vi "test2.vi"() -> ()   [LabVIEW 2017]
uses:
  <userlib>/_NEVSTOP/Communicable State Machine(CSM)/AdvanceAPI/CSM - Revert Arguments-Safe String.vi
  <userlib>/_NEVSTOP/Communicable State Machine(CSM)/_Shared/Trim Single-line Text.vi
  <userlib>/_NEVSTOP/Communicable State Machine(CSM)/AdvanceAPI/CSM - Make String Arguments Safe.vi
  <userlib>/_NEVSTOP/Communicable State Machine(CSM)/AdvanceAPI/CSM - Break Down Multiple States String.vi
  <userlib>/_NEVSTOP/Communicable State Machine(CSM)/AdvanceAPI/CSM - Compact Multiple States.vi
  <userlib>/_NEVSTOP/Communicable State Machine(CSM)/AdvanceAPI/CSM - Keywords.vi
  <userlib>/_NEVSTOP/Communicable State Machine(CSM)/_Polymophic/CSM - Filter Duplicated Lines.vi
  <userlib>/_NEVSTOP/Communicable State Machine(CSM)/Communicable State Machine.lvlib
  ad7296c1-f9ce-49fc-bda0-69987307e577.vi
  bdc5c617-8b58-41cb-8bd3-c5aaa467307a.vi
  <userlib>/_NEVSTOP/Communicable State Machine(CSM)/addons/MassData-Parameter/CSM MassData Parameter Support.lvlib
  <userlib>/_NEVSTOP/Communicable State Machine(CSM)/_Polymophic/Build No-Reply Asynchronous Message with Arguments.vi
panel:
  out "Found":bool
  out "Waited(ms) 2":u32
  out "Waited(ms)":u32
  out "error out":errorcluster
  out "A 4":bool=TRUE
  in  "停止":bool
  in  "布尔":bool
  out "A 3":bool=TRUE
  out "A 2":bool=TRUE
  out "A 1":bool=TRUE
  out "Error Occurred":errorcluster
  out "State History":string
  in  "Name (\"\" to Use UUID)":string="test2"
  in  "Slide":dbl(slide) caption="Flood of Events:\n\nPanel/Pane Size Event\nSlide/Knob... User Event by dragging\nNumeric Control Value Change Event by Arraw Button" scale=0.0..10.0
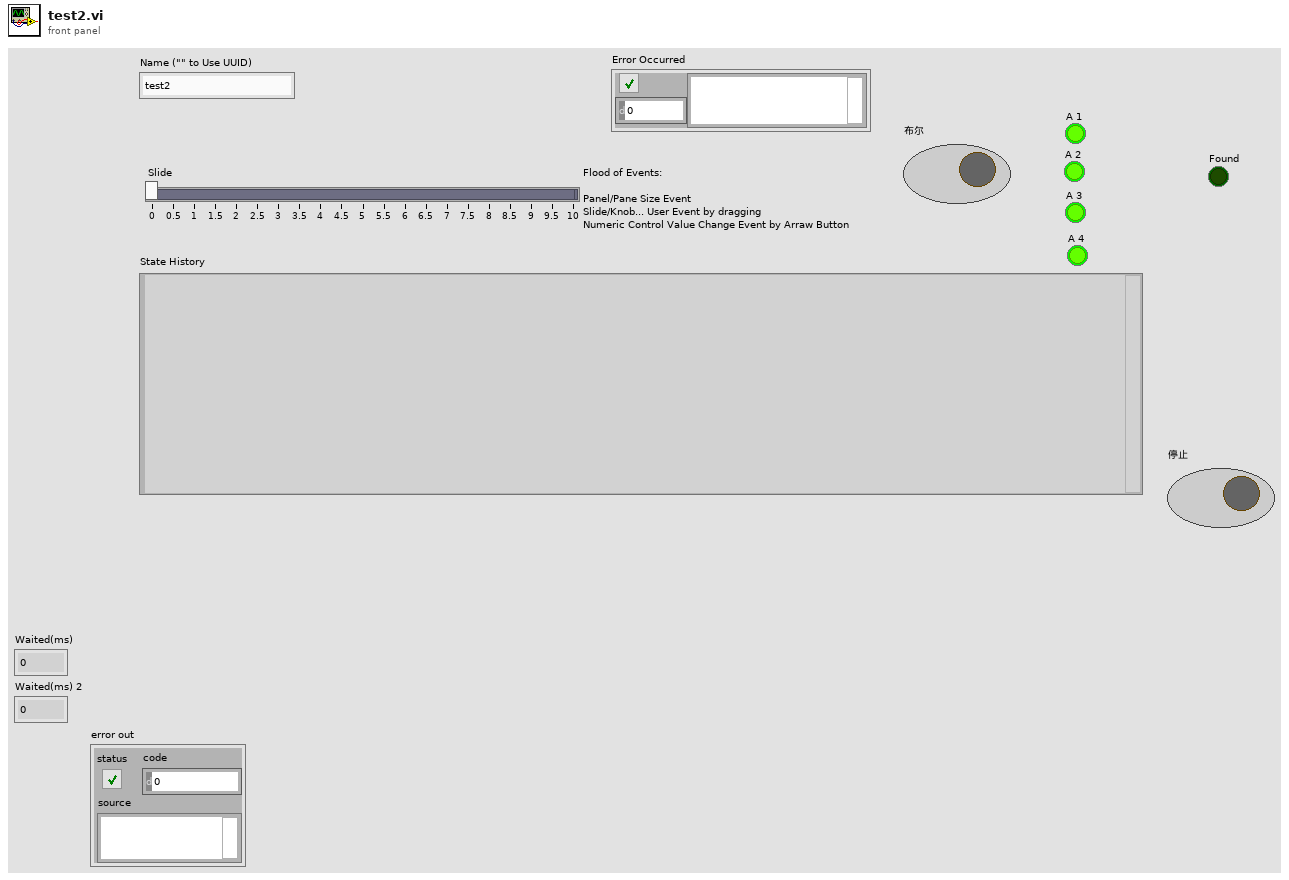
[diagram p1: front panel]
types:
  T1 = enum32{"Invalid", "Standard", "Closed", "Hidden", "Minimized", "Maximized"}
  T2 = enum32{"invalid app kind", "Development System", "Run Time System", "Student Edition", "Embedded LabVIEW", "Evaluation", "Custom"}
  T3 = typedef "Communicable State Machine.lvlib/_CSM_Response Source Message.ctl" = cluster{"‘State":string, "’Arguments":string, "’Error":errorcluster}
  T4 = cluster{"Current VI Reference":refnum<vi>, "Close Panel on Exit?":bool}
  T5 = cluster{"Core":cluster{"Current VI Reference":refnum<vi>, "Close Panel on Exit?":bool}, "Your Boolean data":bool, "Your string data":string}
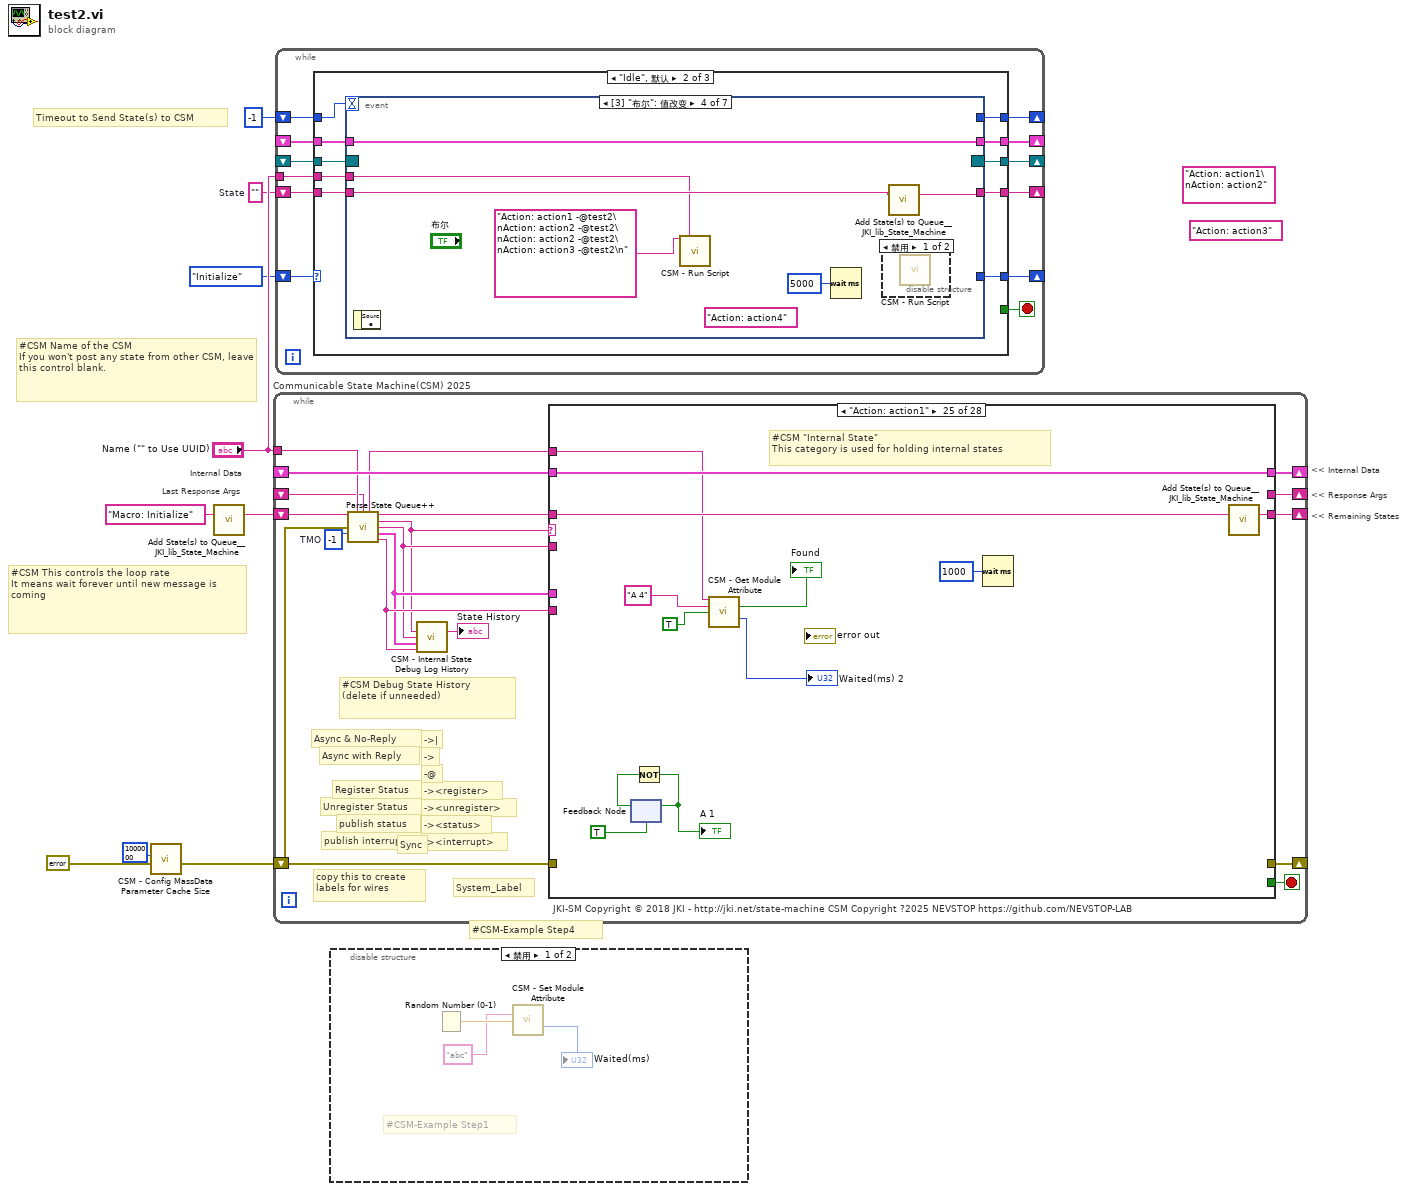
[diagram p0: block diagram]
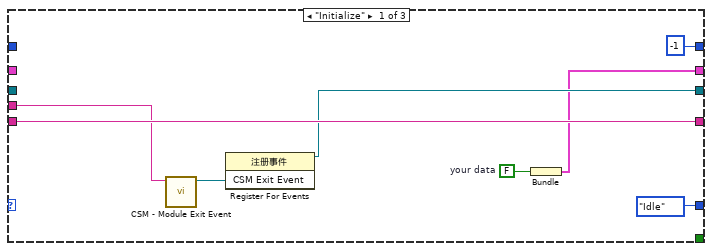
[diagram p3: hidden frame]
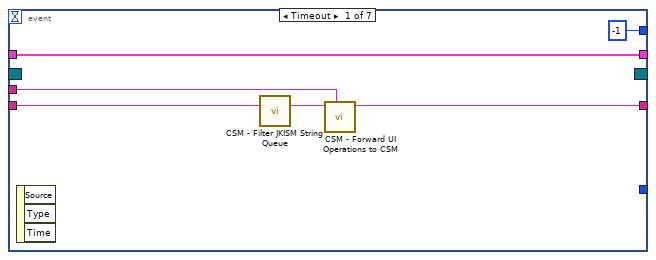
[diagram p4: hidden frame]
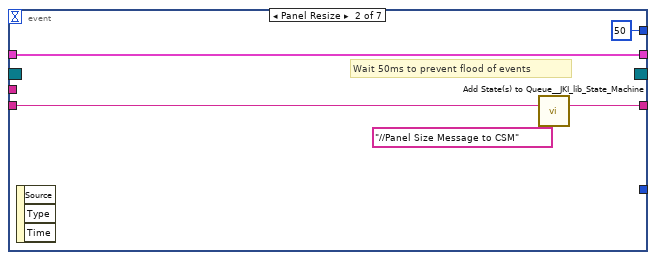
[diagram p5: hidden frame]
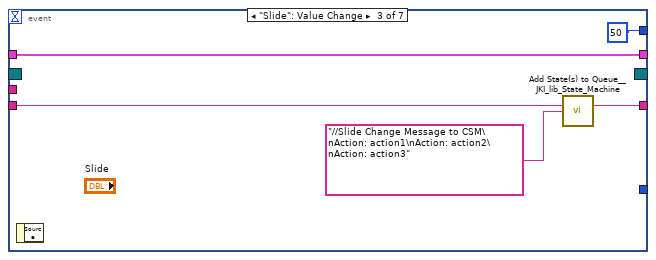
[diagram p6: hidden frame]
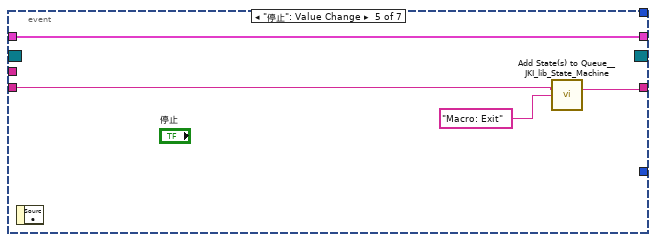
[diagram p8: hidden frame]
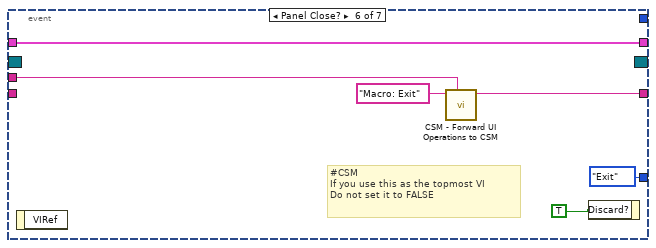
[diagram p9: hidden frame]
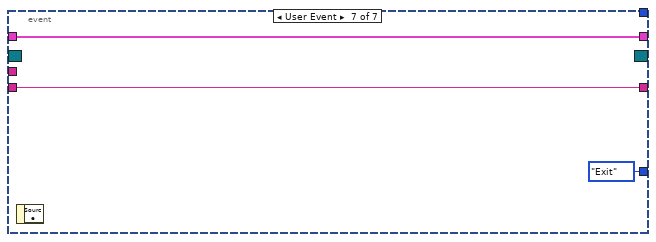
[diagram p10: hidden frame]
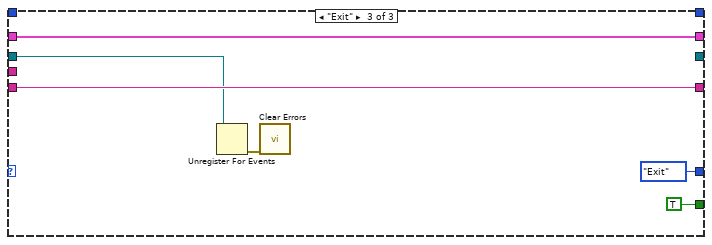
[diagram p11: hidden frame]
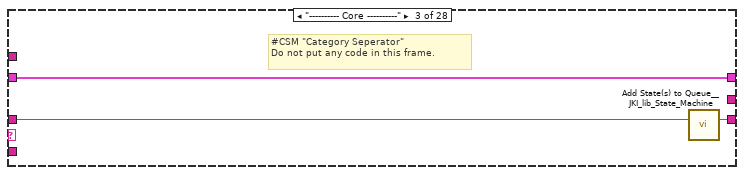
[diagram p14: hidden frame]
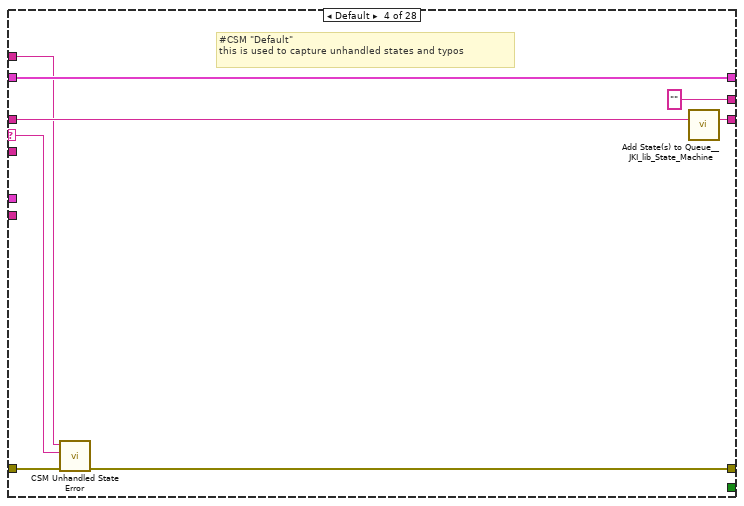
[diagram p15: hidden frame]
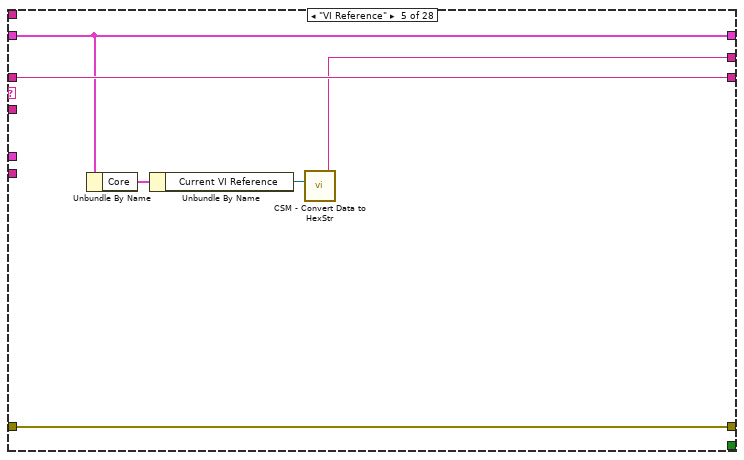
[diagram p16: hidden frame]
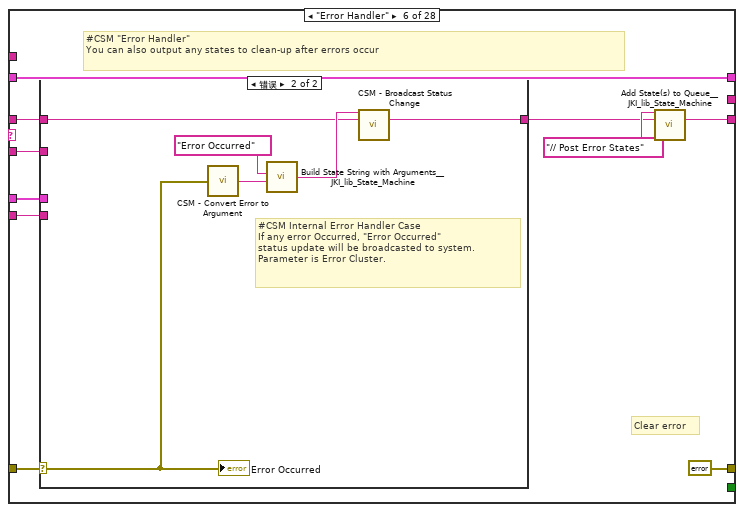
[diagram p17: hidden frame]
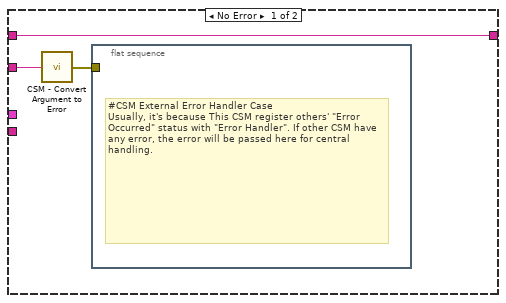
[diagram p18: hidden frame]
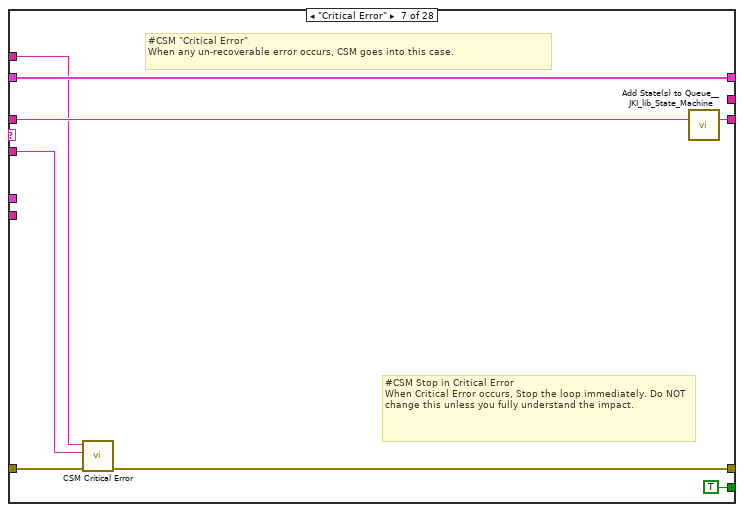
[diagram p19: hidden frame]
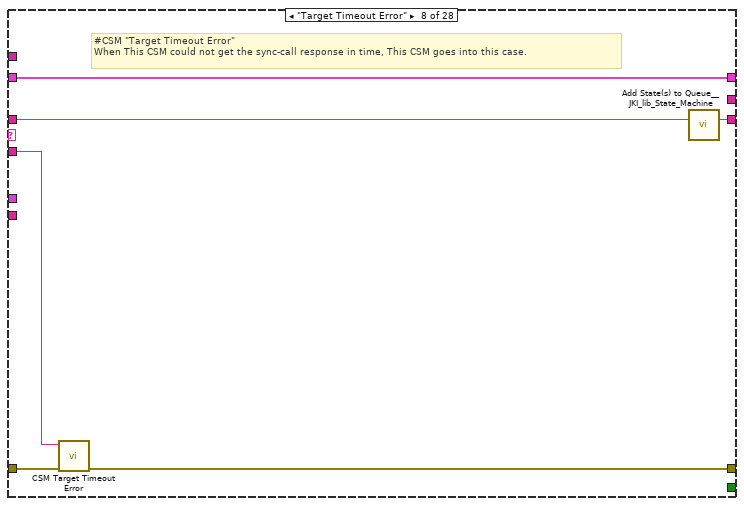
[diagram p20: hidden frame]
diagram:
  (unwired) "Action: action3" ("State(s) in Front (\"\")")
  (unwired) "Action: action1\nAction: action2" ("State(s) at Back (\"\")")
  w7 = ""  # State
  # "#CSM-Example Step4"
  # "Timeout to Send State(s) to CSM"
  # "Last Response Args"
  # "Internal Data"
  # "#CSM Name of the CSM\nIf you won't post any state from other CSM, leave this control blank."
  # "#CSM This controls the loop rate\nIt means wait forever until new message is coming"
  # "<< Internal Data"
  # "<< Response Args"
  # "<< Remaining States"
  n1 = call <userlib>:"CSM - Config MassData Parameter Cache Size.vi"("Error in"=errorcluster {"status"=FALSE, "code"=0, "source"=""} ("error out"), "Size (50M)"=1000000 ("size(1M)")) -> ("Error out"=w1:errorcluster)  [unwired: 9 in]
  n2 = call <vilib>:"Add State(s) to Queue__JKI_lib_State_Machine.vi"("State(s) in (\"\")"="Macro: Initialize" ("Init State(\"Macro: Initialize\")")) -> ("States Out"=w4:string)  [unwired: 14 in]
  n3 = while "Communicable State Machine(CSM) 2025" {
    shift-right: [w22] -> _
    shift-left: _ -> [w21]
    shift-right: [w25] -> _
    shift-left: w1 -> [w11]
    shift-right: [w24] -> _
    shift-left: w4 -> [w26]
    tunnel: "Name (\"\" to Use UUID)" -> [w18]
    shift-right: [w19] -> _
    shift-left: _ -> [w13]
    stop <- w23 stop-if-true
    w20 = -1  # TMO
    # "#CSM Debug State History\n(delete if unneeded)"
    # "-><interrupt>"
    # "-><status>"
    # "-><unregister>"
    # "-><register>"
    # "-@"
    # "->"
    # "->|"
    # "publish interrupt"
    # "publish status"
    # "Unregister Status"
    # "Register Status"
    # "Sync"
    # "Async with Reply"
    # "Async & No-Reply"
    # "JKI-SM Copyright © 2018 JKI - http://jki.net/state-machine CSM Copyright ?2025 NEVSTOP https://github.com/NEVSTOP-LAB"
    # "copy this to create labels for wires"
    # "System_Label"
    n4 = call <userlib>:"Parse State Queue++.vi"("State Queue"=w26, "Name (\"\" to Use UUID)"=w18, "Response Arguments"=w13, "Previous Error"=w11, "Dequeue (1 ms)"=w20) -> ("Name Used"=w12:string, "Remaining States"=w27:string, "Current State"=w14:string, "Arguments"=w15:string, "Additional Information"=w16:T3, "Source CSM"=w17:string)  [unwired: 5 in]
    n5 = call <userlib>:"CSM - Internal State Debug Log History.vi"("State"=w14, "Arguments (\"\")"=w15, ">> Response Source Message >>"=w16, "Source (\"\")"=w17) -> ("Debug Log"=→"State History":string)  [unwired: 11 in]
    n6 = case shown="\"Action: action1\"" w14 {
      selector: w14 -> [_ _ _ w38 _ _ _ _ _ _ _ _ _ _ _ _ _ _ _ _ _ _ _ _ _ _ _ _]
      tunnel: w27 -> [w28 w31 w34 w42 w47 w52 w75 w81 w87 w97 w104 w116 w120 w123 w129 w131 w137 w140 w144 w150 w152 w155 w159 w164 w176 w183 w190 w215]
      tunnel: w15 -> [_ _ _ _ _ w51 w71 w78 w84 w91 _ _ _ _ _ _ _ _ _ _ _ _ w157 _ _ _ _ _]
      tunnel: w21 -> [w29 w30 w32 w40 w46 w57 w73 w79 w85 w95 w103 w110 w118 w121 _ w130 w132 w138 w142 w148 w151 w154 w158 w162 w174 w181 w188 w213]
      tunnel: [_ _ _ w35 w48 errorcluster {"status"=FALSE, "code"=0, "source"=""} ("error out") w68 w76 w82 w98 _ _ _ _ _ _ w133 _ _ _ _ _ _ _ _ _ _ _] -> w25
      tunnel: w11 -> [_ _ _ w36 w48 w55 w69 w77 w83 _ _ _ _ _ _ _ w134 _ _ _ _ _ _ _ _ _ _ _]
      tunnel: [w28 w31 w33 w41 w47 w53 w74 w80 w86 w96 w104 w115 w119 w122 w128 w131 w136 w139 w143 w149 w152 w155 w159 w163 w175 w182 w189 w214] -> w24
      tunnel: [_ _ _ _ _ _ TRUE _ _ _ _ _ TRUE _ _ _ _ _ _ _ _ _ _ _ _ _ _ _] -> w23
      tunnel: [w29 w30 w32 w40 w46 w57 w73 w79 w85 w94 w103 w114 w118 w121 w127 w130 w132 w138 w142 w148 w151 w154 w158 w162 w174 w181 w188 w213] -> w22
      tunnel: w17 -> [_ _ _ _ _ w50 _ _ _ w92 _ _ _ _ _ _ _ _ _ _ _ _ _ _ _ _ _ _]
      tunnel: w16 -> [_ _ _ _ _ w49 _ _ _ w93 _ _ _ _ _ _ _ _ _ _ _ _ _ _ _ _ _ _]
      tunnel: [_ _ _ "" w43 _ _ _ _ _ _ _ _ _ _ _ _ _ _ _ _ "API1 Response" w156 _ _ _ _ _] -> w19
      tunnel: w12 -> [_ _ _ w37 _ _ w70 _ _ _ _ _ _ _ _ _ _ _ _ _ _ _ _ _ w167 _ _ _]
      frame "", "Idle" {
        # "#CSM \"Idle/Event Handler\"\nexecutes when the state queue is empty"
      }
      frame "CSM Documentation" {
        # "#CSM State Syntax\n\n// Comment line, all text to the right of “//” will be ignored\n// Local Message Example\nDoSth: DoA >> Arguments\n\n// Sync Call Example\nAPI: xxxx >> Arguments -@ TargetModule\n\n// Async Call Example\nAPI: xxxx >> Arguments -> TargetModule\n\n// Async Call without Reply Example\nAPI: xxxx >> Arguments ->| TargetModule\n\n// Broadcast normal status:\nStatus >> StatusArguments  -><status>\n\n// Broadcast Interrupt status:\nInterrupt >> StatusArguments  -><interrupt>\n\n// Register Source Module's status to Handler Module\nStatus@Source Module >> Handler Module@Handler Module -><register>\n\n// Unegister Source Module's status\nStatus@Source Module >> Handler Module -><unregister>"
        # "#CSM README FIRST\n\nCommunicable State Machine(CSM) is a LabVIEW application framework that builds upon JKI State Machine(JKISM). It follows the pattern of JKISM and extends the keywords to describe message communication between modules, including concepts such as Sync-Message, Async-Message, Subscription/Unsubscription of status - essential elements for creating reusable code modules. For more information, please visit the CSM wiki: https://nevstop-lab.github.io/CSM-Wiki/\n\nFor instructions on JKI State Machine, visit: \n    http://jki.net/state-machine/\nFor information about CSM, visit: \n    https://github.com/NEVSTOP-LAB"
        # "#CSM \"Documentation\"\nCase for holding CSM Documenation"
      }
      frame "---------- Core ----------" {
        # "#CSM \"Category Seperator\"\nDo not put any code in this frame."
        n7 = call <vilib>:"Add State(s) to Queue__JKI_lib_State_Machine.vi"("State(s) in (\"\")"=w34) -> ("States Out"=w33:string)  [unwired: 14 in]
      }
      frame Default {
        # "#CSM \"Default\"\nthis is used to capture unhandled states and typos"
        n8 = call <userlib>:"CSM Unhandled State Error.vi"("error in (no error)"=w36, "Undefined State"=w38, "CSM Name"=w37) -> ("error out"=w35:errorcluster)  [unwired: 8 in]
        n9 = call <vilib>:"Add State(s) to Queue__JKI_lib_State_Machine.vi"("State(s) in (\"\")"=w42) -> ("States Out"=w41:string)  [unwired: 14 in]
      }
      frame "VI Reference" {
        n10 = Unbundle By Name(w46) -> ("Core"=w45:T4)
        n11 = Unbundle By Name(w45) -> ("Current VI Reference"=w44:refnum<vi>)
        n12 = call <userlib>:"CSM - Convert Data to HexStr.vi"("Variant"=w44) -> ("HEX String (0-9,A-F)"=w43:string)  [unwired: 8 in]
      }
      frame "Error Handler" {
        # "#CSM \"Error Handler\"\nYou can also output any states to clean-up after errors occur"
        # "Clear error"
        n13 = case shown="错误" w55 {
          selector: w55 -> [_ w62]
          tunnel: [w61 w64] -> w54
          tunnel: w52 -> [w61 w63]
          tunnel: w51 -> [w60 _]
          tunnel: w50 -> [_ _]
          tunnel: w49 -> [_ _]
          frame No Error {
            n14 = call <userlib>:"CSM - Convert Argument to Error.vi"("Argument"=w60) -> ("Error"=w59:errorcluster)  [unwired: 4 in]
            n15 = flat-sequence {
              tunnel: w59 -> [_]
              frame #0 {
                # "#CSM External Error Handler Case\nUsually, it's because This CSM register others' \"Error Occurred\" status with \"Error Handler\". If other CSM have any error, the error will be passed here for central handling."
              }
            }
          }
          frame Error {
            # "#CSM Internal Error Handler Case \nIf any error Occurred, \"Error Occurred\" \nstatus update will be broadcasted to system.\nParameter is Error Cluster."
            n16 = call <userlib>:"CSM - Convert Error to Argument.vi"("Error"=w62) -> ("Argument"=w66:string)  [unwired: 4 in]
            n17 = call <vilib>:"Build State String with Arguments__JKI_lib_State_Machine.vi"("Arguments (\"\")"=w66, "State"="Error Occurred" ("Status with Arguments")) -> ("State with Arguments"=w65:string)  [unwired: 4 in]
            n18 = call <userlib>:"CSM - Broadcast Status Change.vi"("Status With Arguments"=w65, "State Queue"=w63) -> ("Remaining States"=w64:string)  [unwired: 13 in]
            "Error Occurred" <- w62
          }
        }
        n19 = call <vilib>:"Add State(s) to Queue__JKI_lib_State_Machine.vi"("State(s) in Front (\"\")"="// Post Error States", "State(s) in (\"\")"=w54) -> ("States Out"=w53:string)  [unwired: 13 in]
      }
      frame "Critical Error" {
        # "#CSM \"Critical Error\"\nWhen any un-recoverable error occurs, CSM goes into this case."
        # "#CSM Stop in Critical Error\nWhen Critical Error occurs, Stop the loop immediately. Do NOT change this unless you fully understand the impact."
        n20 = call <userlib>:"CSM Critical Error.vi"("error in (no error)"=w69, "Arugments (As Reason)"=w71, "CSM Name"=w70) -> ("error out"=w68:errorcluster)  [unwired: 8 in]
        n21 = call <vilib>:"Add State(s) to Queue__JKI_lib_State_Machine.vi"("State(s) in (\"\")"=w75) -> ("States Out"=w74:string)  [unwired: 14 in]
      }
      frame "Target Timeout Error" {
        # "#CSM \"Target Timeout Error\"\nWhen This CSM could not get the sync-call response in time, This CSM goes into this case."
        n22 = call <userlib>:"CSM Target Timeout Error.vi"("error in (no error)"=w77, "Arguments (As CSM Name)"=w78) -> ("error out"=w76:errorcluster)  [unwired: 9 in]
        n23 = call <vilib>:"Add State(s) to Queue__JKI_lib_State_Machine.vi"("State(s) in (\"\")"=w81) -> ("States Out"=w80:string)  [unwired: 14 in]
      }
      frame "Target Error" {
        # "#CSM \"Target Error\"\nWhen This CSM try to communicate with an un-existed CSM, This CSM goes into this case."
        n24 = call <userlib>:"CSM Target Error.vi"("error in (no error)"=w83, "Arguments (As CSM Name)"=w84) -> ("error out"=w82:errorcluster)  [unwired: 9 in]
        n25 = call <vilib>:"Add State(s) to Queue__JKI_lib_State_Machine.vi"("State(s) in (\"\")"=w87) -> ("States Out"=w86:string)  [unwired: 14 in]
      }
      frame "Async Response", "Response" {
        n26 = Unbundle(w93) -> ("‘State"=w90:string, "’Arguments"=w89:string, "’Error"=w88:errorcluster)
        n27 = case shown="默认" w90 {
          tunnel: [w99] -> w96
          tunnel: w97 -> [w100]
          tunnel: [w102] -> w94
          tunnel: w95 -> [w102]
          tunnel: [w101] -> w98
          tunnel: w88 -> [w101]
          tunnel: w92 -> [_]
          tunnel: w91 -> [_]
          tunnel: w89 -> [_]
          frame 默认 {
            # "#CSM \"Async Response\"\nHandle Async-call Response (\"Async Response\" for ->)"
            # "#CSM \"Response\"\nHandle Sync-call Response (\"Response\" for -@)"
            # "#CSM Response Comments\nAfter Message is executed, CSM goes to this state for receive the response.\n    For Async Message(->), \"Async Response\" is used. This CSM will goes to \"Async Message Posted\" immediately and receive the \"Async Response\" after the callee finishes the message.\n    For Sync Message(@),  This CSM will wait until the message is done and immediately goes to \"Response\""
            n28 = call <vilib>:"Add State(s) to Queue__JKI_lib_State_Machine.vi"("State(s) in (\"\")"=w100) -> ("States Out"=w99:string)  [unwired: 14 in]
          }
        }
      }
      frame "Async Message Posted" {
        # "#CSM \"Async Message Posted\"\nAfter Async Message is posted (-> or ->| ), CSM goes to this state for post-action.\nYou can use Argument - State to tell which Async Message is called."
      }
      frame "Initialize Core Data" {
        # "#CSM \"Initialize Core Data\"\nThis is used to determine panel behavior on exit"
        # "originally closed?"
        # "exe?"
        # "If panel starts closed or is an EXE, then close it when we exit"
        n29 = property class="VI"() -> ("FP.State"=w107:T1)  [unwired: 2 in, 2 out]
        n30 = property class="App"() -> ("App.Kind"=w113:T2)  [unwired: 2 in, 2 out]
        n31 = control-ref of="Current VI Reference"() -> (w108:refnum<vi>)
        n32 = Equal?(x=w107, y=T1."Closed" ("Front Panel Window:State")) -> (x = y?=w105:bool)
        n33 = Equal?(x=w113, y=T2."Run Time System" ("Application:Kind")) -> (x = y?=w111:bool)
        n34 = Or(x=w105, y=w111) -> (x .or. y?=w109:bool)
        n35 = Bundle By Name(cluster=w110, "Core.Current VI Reference"=w108, "Core.Close Panel on Exit?"=w109) -> (w114:T5)
        n36 = call <vilib>:"Add State(s) to Queue__JKI_lib_State_Machine.vi"("State(s) in (\"\")"=w116) -> ("States Out"=w115:string)  [unwired: 14 in]
      }
      frame "Exit" {
        # "#CSM \"Exit\"\nCase for exiting the loop. No errors that occur here will be handled."
        n37 = call <vilib>:"Add State(s) to Queue__JKI_lib_State_Machine.vi"("State(s) in (\"\")"=w120) -> ("States Out"=w119:string)  [unwired: 14 in]
      }
      frame "---------- Data ----------" {
        # "#CSM \"Category Seperator\"\nDo not put any code in this frame."
        n38 = call <vilib>:"Add State(s) to Queue__JKI_lib_State_Machine.vi"("State(s) in (\"\")"=w123) -> ("States Out"=w122:string)  [unwired: 14 in]
      }
      frame "Data: Initialize" {
        w124 = T4 {"Current VI Reference"=refnum, "Close Panel on Exit?"=FALSE}  # Core
        w126 = TRUE  # Your Boolean data
        w125 = ""  # Your string data
        # "#CSM \"Data: Initialize\"\nInitialize the shift-register data, here.\n(data names are defined by what you wire into the bundle function)"
        # "#CSM do not delete - used by framework"
        # "#CSM Expand Bundle to add new data elements to shift register data."
        # "#CSM Add new data here."
        # "#CSM Data names and types of shift register data are defined by this bundle."
        n39 = Bundle("Core"=w124, "Your Boolean data"=w126, "Your string data"=w125) -> (w127:T5)  [unwired: 1 in]
        n40 = call <vilib>:"Add State(s) to Queue__JKI_lib_State_Machine.vi"("State(s) in (\"\")"=w129) -> ("States Out"=w128:string)  [unwired: 14 in]
      }
      frame "Data: Update Indicators" {
      }
      frame "Data: Cleanup" {
        # "#CSM \"Data: Cleanup\"\nCleanup any data and references, here.\n(this is called automatically, by the Macro: Exit)"
        n41 = Unbundle By Name(w132) -> ("Core.Current VI Reference"=w135:refnum<vi>)
        n42 = Close Reference(reference=w135, error in (no error)=w134) -> (error out=w133:errorcluster)
        n43 = call <vilib>:"Add State(s) to Queue__JKI_lib_State_Machine.vi"("State(s) in (\"\")"=w137) -> ("States Out"=w136:string)  [unwired: 14 in]
      }
      frame "---------- Macro ----------" {
        # "#CSM \"Category Seperator\"\nDo not put any code in this frame."
        n44 = call <vilib>:"Add State(s) to Queue__JKI_lib_State_Machine.vi"("State(s) in (\"\")"=w140) -> ("States Out"=w139:string)  [unwired: 14 in]
      }
      frame "Macro: Initialize" {
        # "#CSM \"Macro: Initialize\"\nInitialization Macro (This is called once, when the VI starts)"
        n45 = call <vilib>:"Add State(s) to Queue__JKI_lib_State_Machine.vi"("State(s) in Front (\"\")"="Data: Initialize\nInitialize Core Data\nData: Update Indicators", "State(s) in (\"\")"=w144) -> ("States Out"=w143:string)  [unwired: 13 in]
      }
      frame "Macro: Exit" {
        # "#CSM \"Macro: Exit\"\nExit Macro (This is called once, when the VI exits)"
        n46 = call <vilib>:"Add State(s) to Queue__JKI_lib_State_Machine.vi"("State(s) in Front (\"\")"="//Exit Sub-Modules ", "State(s) at Back (\"\")"="Data: Cleanup\nExit") -> ("States Out"=w146:string)  [unwired: 13 in]
        n47 = call <vilib>:"Add State(s) to Queue__JKI_lib_State_Machine.vi"("State(s) in Front (\"\")"=w146, "State(s) in (\"\")"=w150) -> ("States Out"=w149:string)  [unwired: 13 in]
      }
      frame "---------- API ----------" {
        # "#CSM \"Category Seperator\"\nDo not put any code in this frame."
      }
      frame "API: API1" {
        # "#CSM API Example\nCopy/Rename this case for your own API"
        # "#CSM >> Source CSM >>\nIf you need to tell who triggered this state , use this string. If it's this case itself, this string is \"\"."
        # "#CSM >> Arguments >>\nDeal with the parameter if any"
        # "#CSM Response\nConnect this to return the response of your API"
      }
      frame "API: API2" {
        # "#CSM API Example\nCopy/Rename this case for your own API"
        # "unpack Hex String  to Variant\nif complex parameter is needed."
        n48 = call <userlib>:"CSM - Convert HexStr to Data.vi"("HEX String"=w157) -> ()  [unwired: 7 in, 2 out]
        n49 = disable-structure shown="Disabled" {
          disable-tunnel: [w160 "API2 Response"] -> w156
          frame Disabled {
            # "pack variant to hexstr \nif complex response is needed."
            # "complex Response"
            n50 = call <userlib>:"CSM - Convert Data to HexStr.vi"() -> ("HEX String (0-9,A-F)"=w160:string)  [unwired: 9 in]
          }
          frame Enabled {
          }
        }
      }
      frame "---------- Action ----------" {
        # "#CSM \"Category Seperator\"\nDo not put any code in this frame."
        n51 = call <vilib>:"Add State(s) to Queue__JKI_lib_State_Machine.vi"("State(s) in (\"\")"=w164) -> ("States Out"=w163:string)  [unwired: 14 in]
      }
      frame "Action: action1" {
        # "#CSM \"Internal State\"\nThis category is used for holding internal states"
        n52 = feedback #1(TRUE) -> (w172:bool)
        n53 = Not(x=w172) -> (.not. x?=w171:bool)
        "A 1" <- w171
        n54 = feedback-in #1(w171) -> ()
        n55 = call <userlib>:"CSM - Get Module Attribute.vi"("CSM Name"=w167, "Attribute"="A 4", "Default Value (Empty Variant)"=TRUE ("A 1")) -> ("Found"=→"Found":bool, "Waited (ms)"=→"Waited(ms) 2":u32)  [unwired: 8 in, 3 out]
        n56 = Wait (ms)(milliseconds to wait=u32 1000 ("等待时间（毫秒）")) -> ()  [unwired: 1 out]
        n57 = call <vilib>:"Add State(s) to Queue__JKI_lib_State_Machine.vi"("State(s) in (\"\")"=w176) -> ("States Out"=w175:string)  [unwired: 14 in]
      }
      frame "Action: action2" {
        # "#CSM \"Internal State\"\nThis category is used for holding internal states"
        n58 = feedback #2(TRUE) -> (w179:bool)
        n59 = Not(x=w179) -> (.not. x?=w178:bool)
        "A 2" <- w178
        n60 = feedback-in #2(w178) -> ()
        n61 = Wait (ms)(milliseconds to wait=u32 1000 ("等待时间（毫秒）")) -> ()  [unwired: 1 out]
        n62 = call <vilib>:"Add State(s) to Queue__JKI_lib_State_Machine.vi"("State(s) in (\"\")"=w183) -> ("States Out"=w182:string)  [unwired: 14 in]
      }
      frame "Action: action3" {
        # "#CSM \"Internal State\"\nThis category is used for holding internal states"
        n63 = disable-structure shown="启用" {
          disable-tunnel: [w200 _] -> _
          frame Disabled {
            w191 = "ymf" ("Target Module (\"\")")
            w207 = cluster{"采集时间":timestamp, "Data":dbl[]} {"采集时间"=timestamp(0 s since 1904-01-01), "Data"=[]}  # Time and Data
            n64 = Random Number (0-1)() -> (number: 0 to 1=w204:dbl)
            n65 = Multiply(x=w204, y=10.0) -> (x*y=w202:dbl)
            n66 = for {
              N: w202 -> [_]
              tunnel: [w208] -> w201 mode=indexing
              n67 = Random Number (0-1)() -> (number: 0 to 1=w208:dbl)
            }
            n68 = Get Date/Time In Seconds() -> (seconds since 1Jan1904=w206:timestamp)
            n69 = Bundle By Name(cluster=w207, "采集时间"=w206, "Data"=w201) -> (w205:cluster{"采集时间":timestamp, "Data":dbl[]})
            n70 = Multiply(x=10.0, y=w201) -> (x*y=w199:dbl[])
            n71 = call "CSM - Convert MassData to Argument.vim"("Data"=w205) -> ("MassData Argument"=w196:string)  [unwired: 7 in, 1 out]
            n72 = call "CSM - Convert MassData to Argument.vim"("Data"=w199) -> ("MassData Argument"=w192:string)  [unwired: 7 in, 1 out]
            n73 = call-poly <userlib>:"Build Message with Arguments++.vi"("State With Arguments"="Action: action1" ("State"), "Arguments (\"\")"=w196, "Target Module (\"\")"=w191) -> ("CSM Message String"=w195:string)  [unwired: 12 in]
            n74 = call-poly <userlib>:"Build Message with Arguments++.vi"("State With Arguments"="Action: action2" ("State"), "Arguments (\"\")"=w192, "Target Module (\"\")"=w191) -> ("CSM Message String"=w193:string)  [unwired: 12 in]
            n75 = call <vilib>:"Add State(s) to Queue__JKI_lib_State_Machine.vi"("State(s) in Front (\"\")"=w193, "State(s) in (\"\")"=w195) -> ("States Out"=w200:string)  [unwired: 13 in]
          }
          frame Enabled {
          }
        }
        n76 = feedback #3(TRUE) -> (w186:bool)
        n77 = Not(x=w186) -> (.not. x?=w185:bool)
        "A 3" <- w185
        n78 = feedback-in #3(w185) -> ()
        n79 = Wait (ms)(milliseconds to wait=u32 1000 ("等待时间（毫秒）")) -> ()  [unwired: 1 out]
        n80 = call <vilib>:"Add State(s) to Queue__JKI_lib_State_Machine.vi"("State(s) in (\"\")"=w190) -> ("States Out"=w189:string)  [unwired: 14 in]
      }
      frame "Action: action4" {
        # "#CSM \"Internal State\"\nThis category is used for holding internal states"
        n81 = feedback #4(TRUE) -> (w211:bool)
        n82 = Not(x=w211) -> (.not. x?=w210:bool)
        "A 4" <- w210
        n83 = feedback-in #4(w210) -> ()
        n84 = Wait (ms)(milliseconds to wait=u32 1000 ("等待时间（毫秒）")) -> ()  [unwired: 1 out]
        n85 = call <vilib>:"Add State(s) to Queue__JKI_lib_State_Machine.vi"("State(s) in (\"\")"=w215) -> ("States Out"=w214:string)  [unwired: 14 in]
      }
    }
  }
  n86 = while {
    shift-right: [w226] -> _
    shift-left: enum16{"Idle", "Initialize", "Exit"}."Initialize" -> [w227]
    tunnel: "Name (\"\" to Use UUID)" -> [w224]
    shift-right: [w222] -> _
    shift-left: w7 -> [w223]
    shift-right: [w220] -> _
    shift-left: -1 -> [w221]
    shift-right: [w219] -> _
    shift-left: _ -> [w218]
    shift-right: [w217] -> _
    shift-left: _ -> [w216]
    stop <- w225 stop-if-true
    n87 = case shown="\"Idle\", 默认" w227 {
      tunnel: [enum16{"Idle", "Initialize", "Exit"}."Idle" w245 enum16{"Idle", "Initialize", "Exit"}."Exit"] -> w226
      tunnel: [_ _ TRUE] -> w225
      tunnel: w224 -> [w231 w244 _]
      tunnel: w223 -> [w234 w242 w284]
      tunnel: [w234 w243 w284] -> w222
      tunnel: w221 -> [_ w240 _]
      tunnel: [-1 w241 _] -> w220
      tunnel: [w230 w238 _] -> w219
      tunnel: w218 -> [_ w239 w283]
      tunnel: [w228 w236 w281] -> w217
      tunnel: w216 -> [_ w237 w281]
      frame "Initialize" {
        w229 = FALSE  # your data
        n88 = call <userlib>:"CSM - Module Exit Event.vi"("Name (\"\" to Use UUID) In"=w231) -> ("CSM Exit Event"=w232:refnum<user-event>)  [unwired: 8 in, 2 out]
        n89 = register-events(w232) -> (reference out=w230:refnum<event-registration>)  [unwired: 2 in, 1 out]
        n90 = Bundle("your data"=w229) -> (w228:cluster{"your data":bool})  [unwired: 1 in]
      }
      frame "Idle", Default {
        n91 = event shown="[3] \"布尔\": 值改变" {
          selector: w239 -> [_ _ _ _ _ _ _]
          dyn-events: [_ _ _ _ _ _ _] -> w238
          timeout: w240 -> [_ _ _ _ _ _ _]
          tunnel: [_ _ _ _ _ enum16{"Idle", "Initialize", "Exit"}."Exit" enum16{"Idle", "Initialize", "Exit"}."Exit"] -> w245
          tunnel: w244 -> [w247 _ _ w262 _ w274 _]
          tunnel: w242 -> [w250 w256 w261 w266 w269 _ w280]
          tunnel: [w248 w255 w260 w265 w268 w273 w280] -> w243
          tunnel: [-1 50 50 _ _ _ _] -> w241
          tunnel: w237 -> [w246 w252 w257 w267 w271 w272 w278]
          tunnel: [w246 w252 w257 w267 w271 w272 w278] -> w236
          event Timeout {
            n92 = event-data() -> ()  [unwired: 1 in, 3 out]
            n93 = call-poly <userlib>:"CSM - Filter JKISM String Queue.vi"("States In"=w250) -> ("States Out"=w249:string)  [unwired: 14 in]
            n94 = call <userlib>:"CSM - Forward UI Operations to CSM.vi"("Name (\"\" to Use UUID)"=w247, "State(s) In (\"\")"=w249) -> ("States Out"=w248:string)  [unwired: 8 in, 1 out]
          }
          event Panel Resize {
            # "Wait 50ms to prevent flood of events"
            n95 = event-data() -> ()  [unwired: 1 in, 3 out]
            n96 = call <vilib>:"Add State(s) to Queue__JKI_lib_State_Machine.vi"("State(s) in (\"\")"=w256, "State(s) at Back (\"\")"="//Panel Size Message to CSM" ("State(s) at Back (\"\")")) -> ("States Out"=w255:string)  [unwired: 13 in]
          }
          event "Slide": Value Change {
            n97 = event-data() -> ()  [unwired: 1 in, 1 out]
            n98 = call <vilib>:"Add State(s) to Queue__JKI_lib_State_Machine.vi"("State(s) in (\"\")"=w261, "State(s) at Back (\"\")"="//Slide Change Message to CSM\nAction: action1\nAction: action2\nAction: action3" ("State(s) at Back (\"\")")) -> ("States Out"=w260:string)  [unwired: 13 in]
          }
          event "布尔": Value Change {
            (unwired) "Action: action4" ("State(s) in Front (\"\")")
            n99 = event-data() -> ()  [unwired: 1 in, 1 out]
            n100 = call <userlib>:"CSM - Run Script.vi"("CSM Scripts"="Action: action1 -@test2\nAction: action2 -@test2\nAction: action2 -@test2\nAction: action3 -@test2\n", "Current Module (\"\" to Generate an ID)"=w262) -> ()  [unwired: 11 in, 3 out]
            n101 = Wait (ms)(milliseconds to wait=u32 5000 ("等待时间（毫秒）")) -> ()  [unwired: 1 out]
            n102 = disable-structure shown="禁用" {
              frame Disabled {
                n103 = call <userlib>:"CSM - Run Script.vi"() -> ()  [unwired: 13 in, 3 out]
              }
              frame Enabled {
              }
            }
            n104 = call <vilib>:"Add State(s) to Queue__JKI_lib_State_Machine.vi"("State(s) in (\"\")"=w266) -> ("States Out"=w265:string)  [unwired: 14 in]
          }
          event "停止": Value Change {
            n105 = event-data() -> ()  [unwired: 1 in, 1 out]
            n106 = call <vilib>:"Add State(s) to Queue__JKI_lib_State_Machine.vi"("State(s) in (\"\")"=w269, "State(s) at Back (\"\")"="Macro: Exit" ("State(s) at Back (\"\")")) -> ("States Out"=w268:string)  [unwired: 13 in]
          }
          event Panel Close? {
            # "#CSM \nIf you use this as the topmost VI\nDo not set it to FALSE"
            n107 = event-data() -> ()  [unwired: 1 in, 1 out]
            n108 = call <userlib>:"CSM - Forward UI Operations to CSM.vi"("Name (\"\" to Use UUID)"=w274, "State(s) In (\"\")"="Macro: Exit" ("State")) -> ("States Out"=w273:string)  [unwired: 8 in, 1 out]
            n109 = event-data("Discard?"=TRUE) -> ()  [unwired: 1 in, 1 out]
          }
          event User Event {
            n110 = event-data() -> ()  [unwired: 1 in, 1 out]
          }
        }
      }
      frame "Exit" {
        n111 = Unregister For Events(event registration refnum=w283) -> (error out=w282:errorcluster)  [unwired: 1 in]
        n112 = call <vilib>:"Clear Errors.vi"("error in (no error)"=w282) -> ()  [unwired: 5 in, 2 out]
      }
    }
  }
  n113 = disable-structure shown="禁用" {
    frame Disabled {
      # "#CSM-Example Step1"
      n114 = Random Number (0-1)() -> (number: 0 to 1=w290:dbl)
      n115 = call <userlib>:"CSM - Set Module Attribute.vi"("Attribute"="abc", "Value"=w290) -> ("CSM Name"=w288:string, "Waited (ms)"=→"Waited(ms)":u32)  [unwired: 9 in, 3 out]
    }
    frame Enabled {
    }
  }
